vi "init.vi"(8 "error in (no error)":errorcluster, 10 "Variant":variant, 11 "USB-6001 in":refnum<class "USB-6001.lvclass">) -> (0 "error out":errorcluster, 3 "USB-6001 out":refnum<class "USB-6001.lvclass">)   [LabVIEW 2025, in "USB IO.lvlib" / "USB-6001.lvclass"]
uses:
  USB-6001.lvclass
  USB-6001.lvclass/USB-6001.ctl
  <vilib>/DAQmx/create/channels.llb/DAQmx Create Channel (DI-Digital Input).vi
  <vilib>/DAQmx/create/channels.llb/DAQmx Create Channel (DO-Digital Output).vi
  USB IO generic/USB IO.lvclass
  <resource>/objmgr/daqmx.rc
panel:
  out "Outputs":tag[](array[tag])
  out "Homing Switch Line":string
  out "DO.Ports":tag[](array[tag])
  out "DO.Lines":tag[](array[tag])
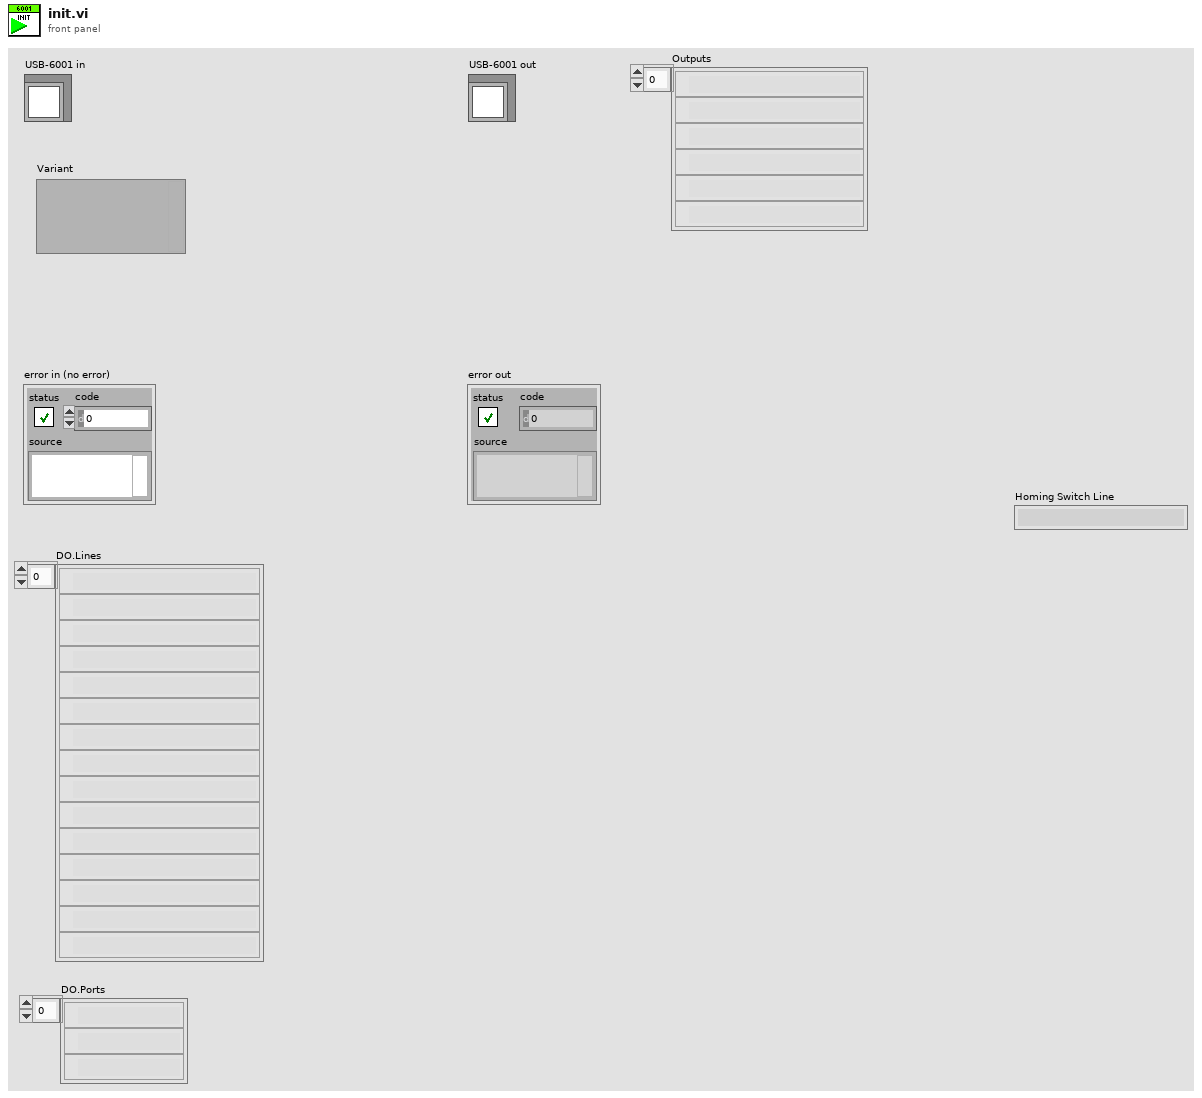
[diagram p1: front panel]
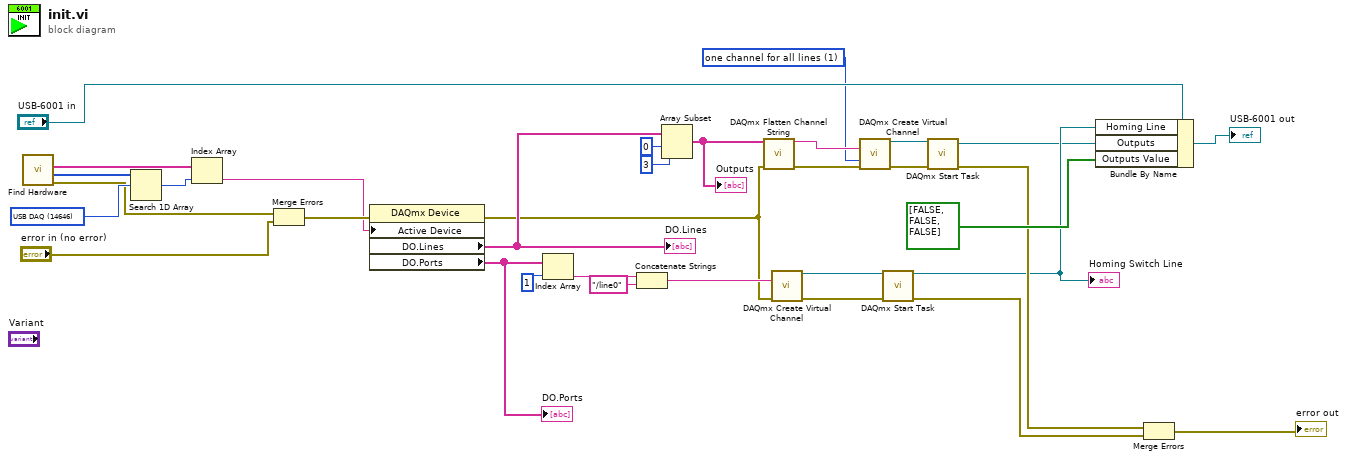
[diagram p0: block diagram]
diagram:
  w13 = 1 items=["one channel for each line", "one channel for all lines"] ("line grouping")
  w32 = 14646 items=["M Series DAQ"=14643, "X Series DAQ"=15858, "E Series DAQ"=14642, "S Series DAQ"=14644, "B Series DAQ"=14662, "SC Series DAQ"=14645, "USB DAQ"=14646, "AO Series"=14647, "Digital I/O"=14648, "TIO Series"=14661, "Dynamic Signal Acquisition"=14649, "Switches"=14650, "CompactDAQ Chassis"=14658, "CompactRIO Chassis"=16144, "C Series Module"=14659, "SCXI Module"=14660, "SCC Connector Block"=14704, "SCC Module"=14705, "NI ELVIS"=14755, "Network DAQ"=14829, "SC Express"=15886, "FieldDAQ"=16151, "TestScale Chassis"=16180, "TestScale Module"=16181, "mioDAQ"=16182, "Unknown"=12588] ("ProductCategory")
  n1 = call "Find Hardware.vi"() -> ("error out"=w27:errorcluster, "Product Category"=w33:i32[], "DevNames"=w30:tag[])  [unwired: 8 in, 1 out]
  n2 = Search 1D Array(1D array=w33, element=w32) -> (index of element=w31:i32)  [unwired: 1 in]
  n3 = Index Array(array=w30, index=w31) -> (element=w26:tag)
  n4 = Merge Errors(w27, "error in (no error)") -> (w29:errorcluster)
  n5 = property class="DAQmx Device"(error in=w29, "Active Device"=w26) -> (error out=w6:errorcluster, "DO.Lines"=w19:tag[], "DO.Ports"=w25:tag[])  [unwired: 1 in, 1 out]
  "DO.Lines" <- w19
  "DO.Ports" <- w25
  n6 = Index Array(array=w25, index=1) -> (element=w23:tag)
  n7 = Concatenate Strings(w23, "/line0" ("string")) -> (w9:string)
  n8 = Array Subset(array=w19, index=0, length=3) -> (w16:tag[])
  "Outputs" <- w16
  n9 = call <vilib>:"DAQmx Flatten Channel String.vi"("names in"=w16, "error in"=w6) -> ("names out"=w14:string, "error out"=w15:errorcluster)  [unwired: 12 in]
  n10 = call-poly <vilib>:"DAQmx Create Virtual Channel.vi"("lines"=w9, "error in"=w6) -> ("task out"=w8:refnum<k21>, "error out"=w7:errorcluster)  [unwired: 12 in]
  n11 = call-poly <vilib>:"DAQmx Create Virtual Channel.vi"("lines"=w14, "line grouping"=w13, "error in"=w15) -> ("task out"=w11:refnum<k21>, "error out"=w12:errorcluster)  [unwired: 11 in]
  n12 = call <vilib>:"DAQmx Start Task.vi"("task/channels in"=w8, "error in"=w7) -> ("task out"=w2:refnum<k21>, "error out"=w3:errorcluster)  [unwired: 12 in]
  "Homing Switch Line" <- w2
  n13 = call <vilib>:"DAQmx Start Task.vi"("task/channels in"=w11, "error in"=w12) -> ("task out"=w1:refnum<k21>, "error out"=w4:errorcluster)  [unwired: 12 in]
  n14 = Bundle By Name(cluster="USB-6001 in", "Homing Line"=w2, "Outputs"=w1, "Outputs Value"=bool[] [FALSE, FALSE, FALSE]) -> (→"USB-6001 out":refnum<class "USB-6001.lvclass">)
  n15 = Merge Errors(w4, w3) -> (→"error out":errorcluster)
